vi "Synth_f_change.vi"(11 "string":string) -> ()   [LabVIEW 2024]
uses:
  Serial Port.vi
  <vilib>/Instr/_visa.llb/VISA Configure Serial Port (Instr).vi
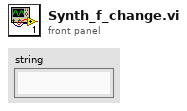
[diagram p1: front panel]
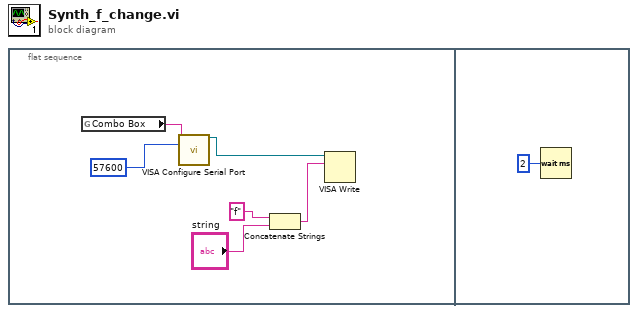
[diagram p0: block diagram]
diagram:
  n1 = flat-sequence {
    frame #0 {
      n2 = global read "Serial Port.vi" "Combo Box"() -> (w1:string)
      n3 = call-poly "VISA Configure Serial Port"("VISA resource name"=w1, "baud rate (9600)"=u32 57600) -> ("VISA resource name out"=w5:refnum<visa-resource-name>)  [unwired: 12 in, 1 out]
      n4 = Concatenate Strings("f", "string") -> (w2:string)
      n5 = VISA Write(VISA resource name=w5, write buffer=w2) -> ()  [unwired: 1 in, 3 out]
    }
    frame #1 {
      n6 = Wait (ms)(milliseconds to wait=u32 2) -> ()  [unwired: 1 out]
    }
  }
